vi "LabviewOscilloscope.vi"() -> ()   [LabVIEW 2014]
uses:
  <vilib>/Instr/_visa.llb/VISA Configure Serial Port (Instr).vi
panel:
  out "ChkSum Error":bool
  out "Sync Error":bool
  out "Timeout Error":bool
  in  "LabviewOscilloscope":T1(tab)=enum."Oscilloscope"
  in  "Voltage Reference":dbl=3.33 caption="V"
  in  "ChkSum":enum16{"ZERO16", "LRC8", "CRC16-CCITT"}(ring)
  in  "Serial Port":T2(ring)
  in  "Baud Rate":u32=9600
  in  "timeout [ms]":u32=100
  in  "SW":u8
  in  "BTN0":bool
  in  "BTN1":bool
  in  "BTN2":bool
  in  "BTN3":bool
  out "FreqSelect":bool
  out "AmplSelect":bool
  out "ShapeSelect":bool=TRUE
  out "Shape1Index":u8
  out "AmplIndex":u8
  out "FreqIndex":u8
  out "Frequency":string="   0,0Hz"
  out "Amplitude":string="   0,00 V"
  out "Shape":string="Const"
  in  "Number of Packets shown":i16=2
  in  "SEND Button":bool
  in  "Record Length":u16=500
  in  "Sample Rate":u16=10000
  out "Oscilloskop":u8[](graph)
  out "XY Graph":cluster{u32[], dbl[]}(graph)
  in  "Start":bool
  out "Raw Packet":string
  out "Raw":string
  # "Received raw data (in hex)"
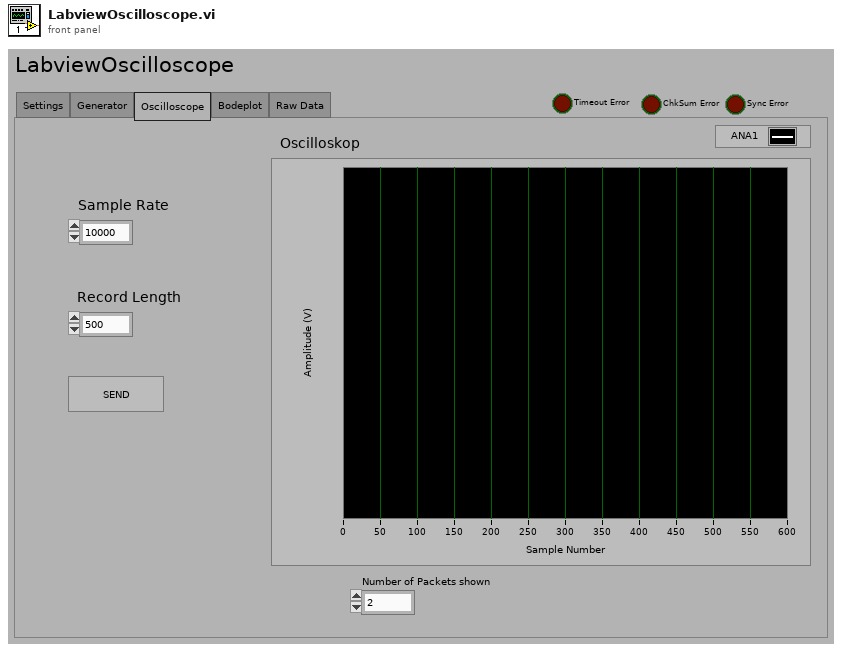
[diagram p1: front panel]
types:
  T1 = enum32{"Settings", "Generator", "Oscilloscope", "Bodeplot", "Raw Data"}
  T2 = enum16{"COM1", "COM2", "COM3", "COM4", "COM5", "COM6", "COM7", "COM8", "COM9", "COM10", "COM11", "COM12", "COM13", "COM14", "COM15", "COM16", "COM17", "COM18", "COM19", "COM20", "COM21", "COM22", "COM23", "COM24", "COM25", "COM26", "COM27", "COM28", "COM29", "COM30"}
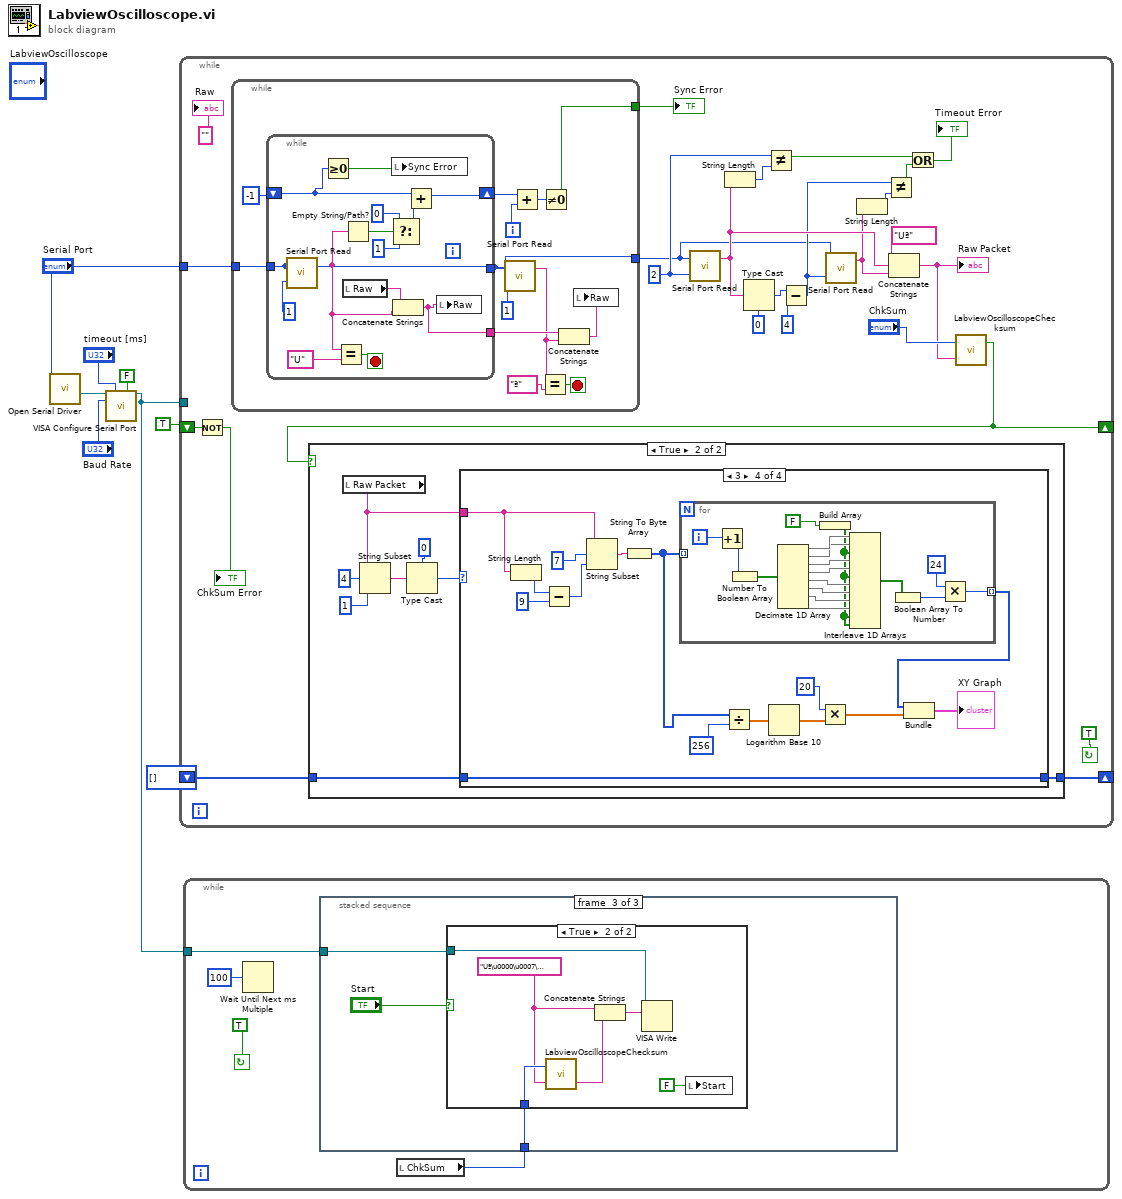
[diagram p0: block diagram]
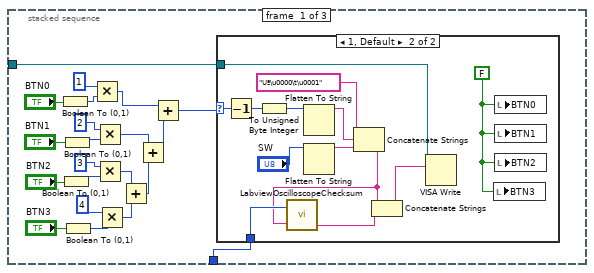
[diagram p2: hidden frame]
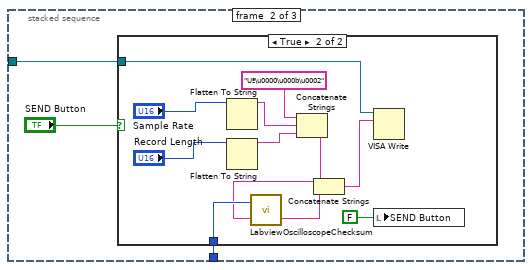
[diagram p4: hidden frame]
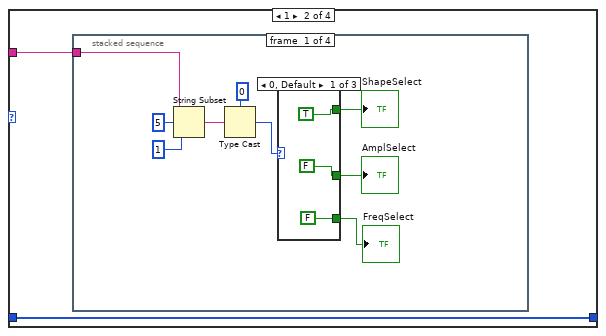
[diagram p9: hidden frame]
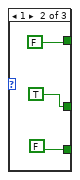
[diagram p10: hidden frame]
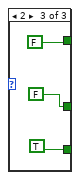
[diagram p11: hidden frame]
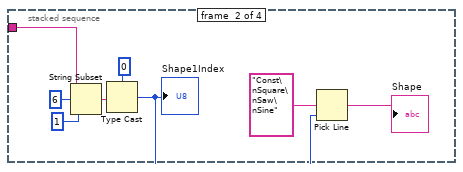
[diagram p12: hidden frame]
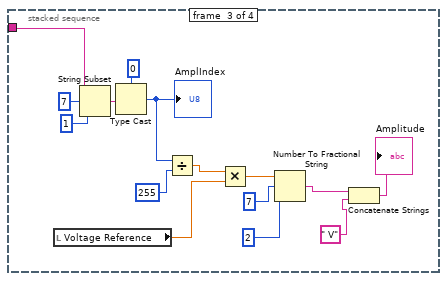
[diagram p13: hidden frame]
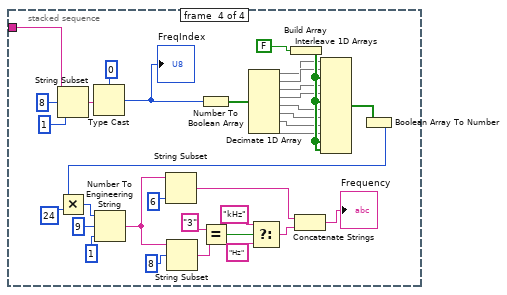
[diagram p14: hidden frame]
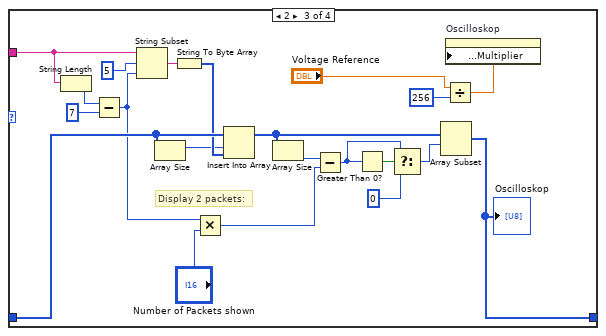
[diagram p15: hidden frame]
diagram:
  n1 = call <vilib>:"Open Serial Driver.vi"("port number"="Serial Port") -> ("output refnum"=w6:refnum<visa-resource-name>)  [unwired: 3 out]
  n2 = call-poly "VISA Configure Serial Port"("VISA resource name"=w6, "timeout (10sec)"="timeout [ms]", "Enable Termination\nChar (T)"=FALSE, "baud rate (9600)"="Baud Rate") -> ("VISA resource name out"=w2:refnum<visa-resource-name>)  [unwired: 10 in, 1 out]
  n3 = while {
    shift-right: [w33] -> _
    shift-left: u8[] [] -> [w32]
    tunnel: "Serial Port" -> [w26]
    shift-right: [w16] -> _
    shift-left: TRUE -> [w15]
    tunnel: w2 -> [_]
    stop <- TRUE continue-if-true
    w13 = 2
    n4 = Not(x=w15) -> (.not. x?=→"ChkSum Error":bool)
    n5 = while {
      tunnel: w26 -> [w186]
      tunnel: [w175] -> w10
      tunnel: [w182] -> w25
      i -> [w179]
      stop <- w185 stop-if-true
      n6 = while {
        tunnel: w186 -> [w189]
        tunnel: [w189] -> w175
        tunnel: [w190] -> w184
        shift-right: [w191] -> w178
        shift-left: -1 -> [w193]
        stop <- w199 stop-if-true
        n7 = call <vilib>:"Serial Port Read.vi"("requested byte count"=1, "port number"=w189) -> ("string read"=w187:string)  [unwired: 1 out]
        n8 = Greater Or Equal To 0?(x=w193) -> (x >= 0?=w192:bool)
        n9 = Equal?(x=w187, y="U") -> (x = y?=w199:bool)
        n10 = Empty String/Path?(string/path=w187) -> (empty?=w194:bool)
        n11 = local read "Raw"() -> (w198:string)
        n12 = Select(t=0, s=w194, f=1) -> (s? t:f=w195:i32)
        n13 = local write "Sync Error"(w192) -> ()
        n14 = Concatenate Strings(w198, w187) -> (w190:string)
        n15 = Add(x=w193, y=w195) -> (x+y=w191:i32)
        n16 = local write "Raw"(w190) -> ()
      }
      n17 = call <vilib>:"Serial Port Read.vi"("requested byte count"=1, "port number"=w175) -> ("string read"=w176:string)  [unwired: 1 out]
      n18 = Add(x=w178, y=w179) -> (x+y=w183:i32)
      n19 = Equal?(x=w176, y="ª") -> (x = y?=w185:bool)
      n20 = Not Equal To 0?(x=w183) -> (x != 0?=w182:bool)
      n21 = Concatenate Strings(w184, w176) -> (w181:string)
      n22 = local write "Raw"(w181) -> ()
    }
    "Sync Error" <- w25
    n23 = call <vilib>:"Serial Port Read.vi"("requested byte count"=w13, "port number"=w10) -> ("string read"=w12:string)  [unwired: 1 out]
    n24 = String Length(string=w12) -> (length=w23:i32)
    n25 = Type Cast(type=i16 0, x=w12) -> (*(type *) &x=w29:i16)
    n26 = Not Equal?(x=w13, y=w23) -> (x != y?=w21:bool)
    n27 = Subtract(x=w29, y=i16 4) -> (x-y=w11:i16)
    n28 = call <vilib>:"Serial Port Read.vi"("requested byte count"=w11, "port number"=w10) -> ("string read"=w9:string)  [unwired: 1 out]
    n29 = String Length(string=w9) -> (length=w24:i32)
    n30 = Not Equal?(x=w11, y=w24) -> (x != y?=w22:bool)
    n31 = Concatenate Strings("Uª", w12, w9) -> (w17:string)
    "Raw Packet" <- w17
    n32 = Or(x=w21, y=w22) -> (x .or. y?=→"Timeout Error":bool)
    n33 = call "LabviewOscilloscopeChecksum.vi"("DATA PACKET"=w17, "ChkSumType"="ChkSum") -> ("Checked"=w16:bool)  [unwired: 1 out]
    n34 = case shown="True" w16 {
      tunnel: [w34 w42] -> w33
      tunnel: w32 -> [w34 w41]
      frame False {
      }
      frame True {
        n35 = local read "Raw Packet"() -> (w37:string)
        n36 = String Subset(string=w37, offset (0)=4, length (rest)=1 ("length (rest)")) -> (substring=w40:string)
        n37 = Type Cast(type=u8 0, x=w40) -> (*(type *) &x=w36:u8)
        n38 = case shown="3" w36 {
          tunnel: w37 -> [_ w45 w122 w151]
          tunnel: [w43 w44 w127 w145] -> w42
          tunnel: w41 -> [w43 w44 w135 w145]
          frame 0, Default {
          }
          frame 1 {
            n39 = stacked-sequence {
              tunnel: w45 -> [w52 w67 w82 w116]
              frame #0 {
                n40 = String Subset(string=w52, offset (0)=5, length (rest)=1 ("length (rest)")) -> (substring=w51:string)
                n41 = Type Cast(type=u8 0, x=w51) -> (*(type *) &x=w49:u8)
                n42 = case shown="0, Default" w49 {
                  tunnel: [TRUE FALSE FALSE] -> w48
                  tunnel: [FALSE TRUE FALSE] -> w47
                  tunnel: [FALSE FALSE TRUE] -> w46
                  frame 0, Default {
                  }
                  frame 1 {
                  }
                  frame 2 {
                  }
                }
                "ShapeSelect" <- w48
                "AmplSelect" <- w47
                "FreqSelect" <- w46
              }
              frame #1 {
                n43 = String Subset(string=w67, offset (0)=6, length (rest)=1 ("length (rest)")) -> (substring=w69:string)
                n44 = Type Cast(type=u8 0, x=w69) -> (*(type *) &x=w65:u8)
                "Shape1Index" <- w65
                n45 = Pick Line(multi-line string="Const\nSquare\nSaw\nSine", line index=w65) -> (output string=→"Shape":string)  [unwired: 1 in]
              }
              frame #2 {
                n46 = local read "Voltage Reference"() -> (w72:dbl)
                n47 = String Subset(string=w82, offset (0)=7, length (rest)=1 ("length (rest)")) -> (substring=w85:string)
                n48 = Type Cast(type=u8 0, x=w85) -> (*(type *) &x=w81:u8)
                "AmplIndex" <- w81
                n49 = Divide(x=w81, y=255) -> (x/y=w79:dbl)
                n50 = Multiply(x=w79, y=w72) -> (x*y=w78:dbl)
                n51 = Number To Fractional String(number=w78, width (-)=7, precision (6)=2) -> (F-format string=w75:string)  [unwired: 1 in]
                n52 = Concatenate Strings(w75, " V") -> (→"Amplitude":string)
              }
              frame #3 {
                n53 = String Subset(string=w116, offset (0)=8, length (rest)=1 ("length (rest)")) -> (substring=w118:string)
                n54 = Type Cast(type=u8 0, x=w118) -> (*(type *) &x=w88:u8)
                "FreqIndex" <- w88
                n55 = Number To Boolean Array(number=w88) -> (Boolean array=w90:bool[])
                n56 = Decimate 1D Array(w90) -> (w91:bool[], w97:bool[], w92:bool[], w98:bool[], w93:bool[], w94:bool[], w95:bool[], w99:bool[])
                n57 = Build Array(FALSE) -> (w100:bool[])
                n58 = Interleave 1D Arrays(w91, w97, w100, w92, w98, w100, w93, w94, w95, w99, w100, w100) -> (w96:bool[])
                n59 = Boolean Array To Number(Boolean array=w96) -> (number=w101:u32)
                n60 = Multiply(x=w101, y=24) -> (x*y=w103:u32)
                n61 = Number To Engineering String(2:1, 3:9, 4:w103) -> (0:w108:string)  [unwired: 1 in]
                n62 = String Subset(string=w108, length (rest)=6) -> (substring=w115:string)  [unwired: 1 in]
                n63 = String Subset(string=w108, offset (0)=8) -> (substring=w113:string)  [unwired: 1 in]
                n64 = Equal?(x="3", y=w113) -> (x = y?=w111:bool)
                n65 = Select(t="kHz", s=w111, f="Hz") -> (s? t:f=w114:string)
                n66 = Concatenate Strings(w115, w114) -> (→"Frequency":string)
              }
            }
          }
          frame 2 {
            # "Display 2 packets:"
            n67 = String Length(string=w122) -> (length=w141:i32)
            n68 = Subtract(x=w141, y=7 ("length (rest)")) -> (x-y=w123:i32)
            n69 = String Subset(string=w122, offset (0)=5, length (rest)=w123) -> (substring=w138:string)
            n70 = Array Size(array=w135) -> (size(s)=w133:i32)
            n71 = String To Byte Array(string=w138) -> (unsigned byte array=w134:u8[])
            n72 = Multiply(x=w123, y="Number of Packets shown") -> (x*y=w125:i32)
            n73 = Insert Into Array(array=w135, index=w133, new element=w134) -> (w128:u8[])
            n74 = Array Size(array=w128) -> (size(s)=w130:i32)
            n75 = Subtract(x=w130, y=w125) -> (x-y=w131:i32)
            n76 = Greater Than 0?(x=w131) -> (x > 0?=w132:bool)
            n77 = Select(t=w131, s=w132, f=0) -> (s? t:f=w126:i32)
            n78 = Array Subset(array=w128, index=w126) -> (w127:u8[])  [unwired: 1 in]
            "Oscilloskop" <- w127
            n79 = Divide(x="Voltage Reference", y=u16 256) -> (x/y=w136:dbl)
            n80 = property on="Oscilloskop" class="WFGraph (strict)"("Y Scale.Offset and Multiplier:Multiplier"=w136) -> ()  [unwired: 2 in, 2 out]
          }
          frame 3 {
            n81 = String Length(string=w151) -> (length=w153:i32)
            n82 = Subtract(x=w153, y=9 ("length (rest)")) -> (x-y=w152:i32)
            n83 = String Subset(string=w151, offset (0)=7, length (rest)=w152) -> (substring=w156:string)
            n84 = String To Byte Array(string=w156) -> (unsigned byte array=w142:u8[])
            n85 = for {
              tunnel: [w159] -> w150 mode=indexing
              tunnel: w142 -> [_] mode=indexing
              i -> [w161]
              n86 = Increment(x=w161) -> (x+1=w160:i32)
              n87 = Number To Boolean Array(number=w160) -> (Boolean array=w172:bool[])
              n88 = Decimate 1D Array(w172) -> (w171:bool[], w165:bool[], w170:bool[], w164:bool[], w169:bool[], w168:bool[], w167:bool[], w163:bool[])
              n89 = Build Array(FALSE) -> (w162:bool[])
              n90 = Interleave 1D Arrays(w171, w165, w162, w170, w164, w162, w169, w168, w167, w163, w162, w162) -> (w166:bool[])
              n91 = Boolean Array To Number(Boolean array=w166) -> (number=w158:u32)
              n92 = Multiply(x=24, y=w158) -> (x*y=w159:u32)
            }
            n93 = Divide(x=w142, y=256) -> (x/y=w144:dbl[])
            n94 = Logarithm Base 10(1:w144) -> (0:w143:dbl[])
            n95 = Multiply(x=20, y=w143) -> (x*y=w146:dbl[])
            n96 = Bundle(w150, w146) -> (→"XY Graph":cluster{u32[], dbl[]})  [unwired: 1 in]
          }
        }
      }
    }
    "Raw" <- ""
  }
  n97 = while {
    tunnel: w2 -> [w202]
    stop <- TRUE continue-if-true
    n98 = Wait Until Next ms Multiple(millisecond multiple=100) -> ()  [unwired: 1 out]
    n99 = local read "ChkSum"() -> (w201:enum16{"ZERO16", "LRC8", "CRC16-CCITT"})
    n100 = stacked-sequence {
      tunnel: w202 -> [w225 w240 w254]
      tunnel: w201 -> [w224 w239 w253]
      frame #0 {
        n101 = Boolean To (0,1)(Boolean="BTN0") -> (0, 1=w219:i16)
        n102 = Boolean To (0,1)(Boolean="BTN2") -> (0, 1=w215:i16)
        n103 = Boolean To (0,1)(Boolean="BTN1") -> (0, 1=w213:i16)
        n104 = Boolean To (0,1)(Boolean="BTN3") -> (0, 1=w217:i16)
        n105 = Multiply(x=u8 1, y=w219) -> (x*y=w211:i16)
        n106 = Multiply(x=u8 2, y=w213) -> (x*y=w209:i16)
        n107 = Multiply(x=u8 3, y=w215) -> (x*y=w207:i16)
        n108 = Multiply(x=u8 4, y=w217) -> (x*y=w208:i16)
        n109 = Add(x=w207, y=w208) -> (x+y=w206:i16)
        n110 = Add(x=w209, y=w206) -> (x+y=w210:i16)
        n111 = Add(x=w211, y=w210) -> (x+y=w205:i16)
        n112 = case shown="1, Default" w205 {
          selector: w205 -> [_ w234]
          tunnel: w225 -> [_ w228]
          tunnel: w224 -> [_ w232]
          frame 0 {
          }
          frame 1, Default {
            w235 = FALSE
            n113 = Decrement(x=w234) -> (x-1=w229:i16)
            n114 = To Unsigned Byte Integer(number=w229) -> (unsigned 8bit integer=w226:u8)
            n115 = Flatten To String(anything=w226) -> (data string=w233:string)  [unwired: 3 in, 2 out]
            n116 = Flatten To String(anything="SW") -> (data string=w236:string)  [unwired: 3 in, 2 out]
            n117 = Concatenate Strings("Uª\u0000\t\u0001", w233, w236) -> (w230:string)
            n118 = call "LabviewOscilloscopeChecksum.vi"("DATA PACKET"=w230, "ChkSumType"=w232) -> ("ChkSum"=w231:string)  [unwired: 1 out]
            n119 = Concatenate Strings(w230, w231) -> (w227:string)
            n120 = VISA Write(VISA resource name=w228, write buffer=w227) -> ()  [unwired: 1 in, 3 out]
            n121 = local write "BTN3"(w235) -> ()
            n122 = local write "BTN0"(w235) -> ()
            n123 = local write "BTN1"(w235) -> ()
            n124 = local write "BTN2"(w235) -> ()
          }
        }
      }
      frame #1 {
        n125 = case shown="True" "SEND Button" {
          tunnel: w240 -> [_ w246]
          tunnel: w239 -> [_ w245]
          frame False {
          }
          frame True {
            n126 = Flatten To String(anything="Sample Rate") -> (data string=w251:string)  [unwired: 3 in, 2 out]
            n127 = Flatten To String(anything="Record Length") -> (data string=w250:string)  [unwired: 3 in, 2 out]
            n128 = Concatenate Strings("Uª\u0000\u000b\u0002", w251, w250) -> (w244:string)
            n129 = call "LabviewOscilloscopeChecksum.vi"("DATA PACKET"=w244, "ChkSumType"=w245) -> ("ChkSum"=w243:string)  [unwired: 1 out]
            n130 = Concatenate Strings(w244, w243) -> (w242:string)
            n131 = VISA Write(VISA resource name=w246, write buffer=w242) -> ()  [unwired: 1 in, 3 out]
            n132 = local write "SEND Button"(FALSE) -> ()
          }
        }
      }
      frame #2 {
        n133 = case shown="True" "Start" {
          tunnel: w254 -> [_ w260]
          tunnel: w253 -> [_ w259]
          frame False {
          }
          frame True {
            w257 = "Uª\u0000\u0007\u0003"
            n134 = call "LabviewOscilloscopeChecksum.vi"("DATA PACKET"=w257, "ChkSumType"=w259) -> ("ChkSum"=w256:string)  [unwired: 1 out]
            n135 = Concatenate Strings(w257, w256) -> (w258:string)
            n136 = VISA Write(VISA resource name=w260, write buffer=w258) -> ()  [unwired: 1 in, 3 out]
            n137 = local write "Start"(FALSE) -> ()
          }
        }
      }
    }
  }
